vi "modbus Ref MCS .vi"() -> (4 "OffCoil":T3, 6 "On Coil":T2, 10 "Temp":T1)   [LabVIEW 2025]
uses:
  <vilib>/Modbus/master/Modbus Master.lvclass
  <vilib>/Analysis/NI_AALBase.lvlib
  <vilib>/Analysis/baseanly.llb/Mean (DBL).vi
  <vilib>/Modbus/master/Create Master Instance (TCP).vi
panel:
  in  "Boolean":bool
  out "TREES AVG array":dbl[](array[numeric])
  out "OD_Right side AVG distributed":dbl format="%0.2f"
  out "ON_Coil AVG distributed":dbl format="%0.2f"
  out "OFF_Coil AVG distributed":dbl format="%0.2f"
  out "AMB RIGHT":dbl[](array[numeric])
  out "ON-COIL 2":dbl[](array[numeric])
  out "OFF-COIL 2":dbl[](array[numeric])
  out "error out":errorcluster
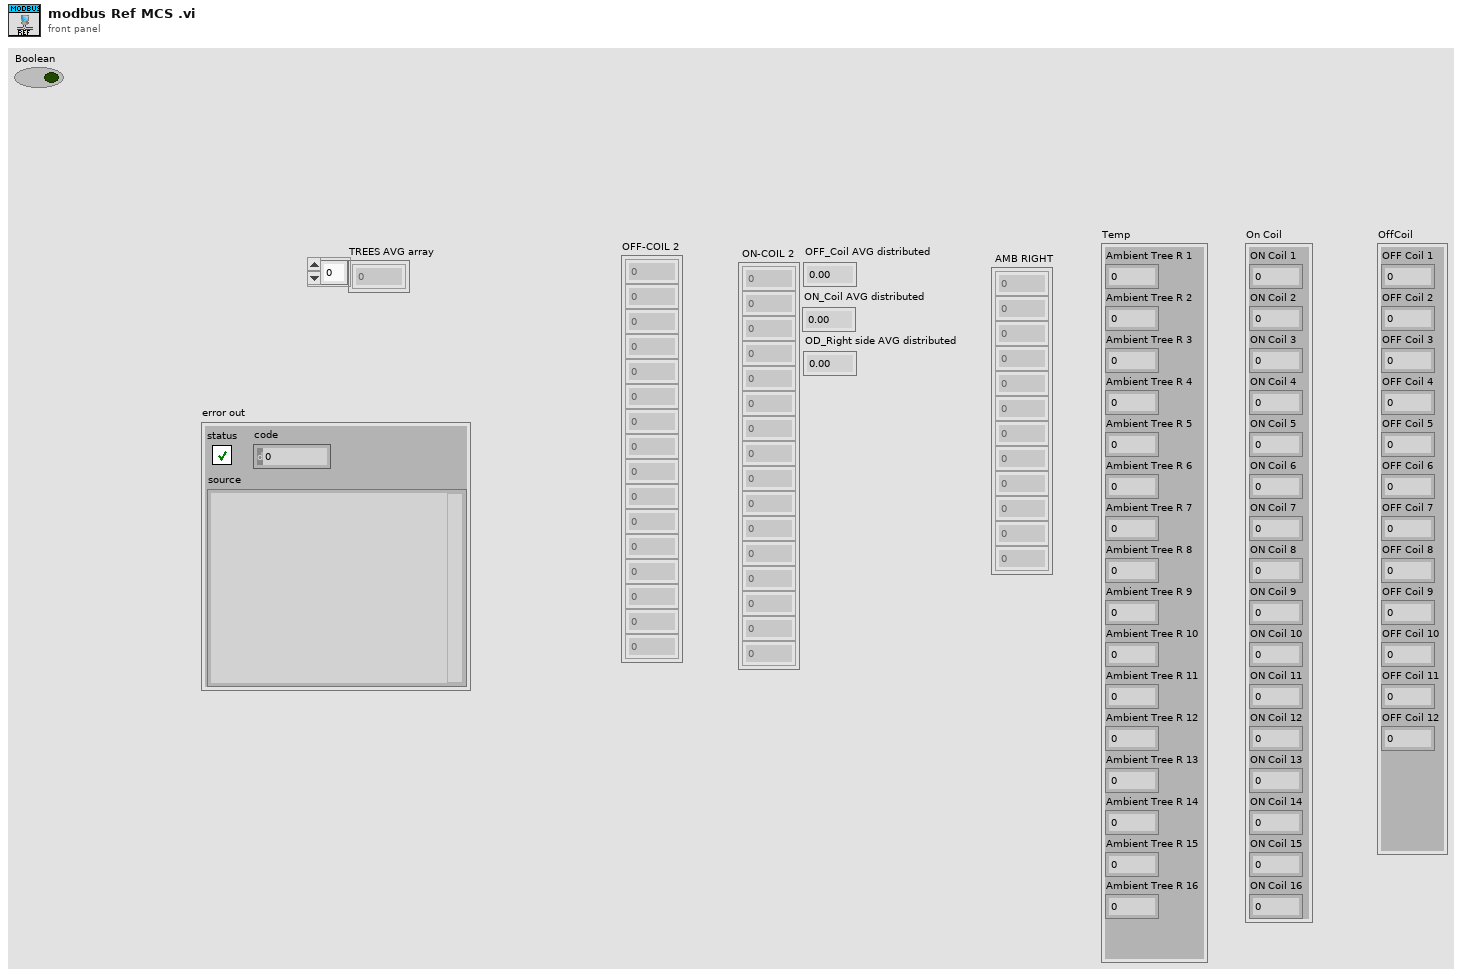
[diagram p1: front panel]
types:
  T1 = cluster{"Ambient Tree R 1":dbl, "Ambient Tree R 2":dbl, "Ambient Tree R 3":dbl, "Ambient Tree R 4":dbl, "Ambient Tree R 5":dbl, "Ambient Tree R 6":dbl, "Ambient Tree R 7":dbl, "Ambient Tree R 8":dbl, "Ambient Tree R 9":dbl, "Ambient Tree R 10":dbl, "Ambient Tree R 11":dbl, "Ambient Tree R 12":dbl, "Ambient Tree R 13":dbl, "Ambient Tree R 14":dbl, "Ambient Tree R 15":dbl, "Ambient Tree R 16":dbl}
  T2 = cluster{"ON Coil 1":dbl, "ON Coil 2":dbl, "ON Coil 3":dbl, "ON Coil 4":dbl, "ON Coil 5":dbl, "ON Coil 6":dbl, "ON Coil 7":dbl, "ON Coil 8":dbl, "ON Coil 9":dbl, "ON Coil 10":dbl, "ON Coil 11":dbl, "ON Coil 12":dbl, "ON Coil 13":dbl, "ON Coil 14":dbl, "ON Coil 15":dbl, "ON Coil 16":dbl}
  T3 = cluster{"OFF Coil 1":dbl, "OFF Coil 2":dbl, "OFF Coil 3":dbl, "OFF Coil 4":dbl, "OFF Coil 5":dbl, "OFF Coil 6":dbl, "OFF Coil 7":dbl, "OFF Coil 8":dbl, "OFF Coil 9":dbl, "OFF Coil 10":dbl, "OFF Coil 11":dbl, "OFF Coil 12":dbl}
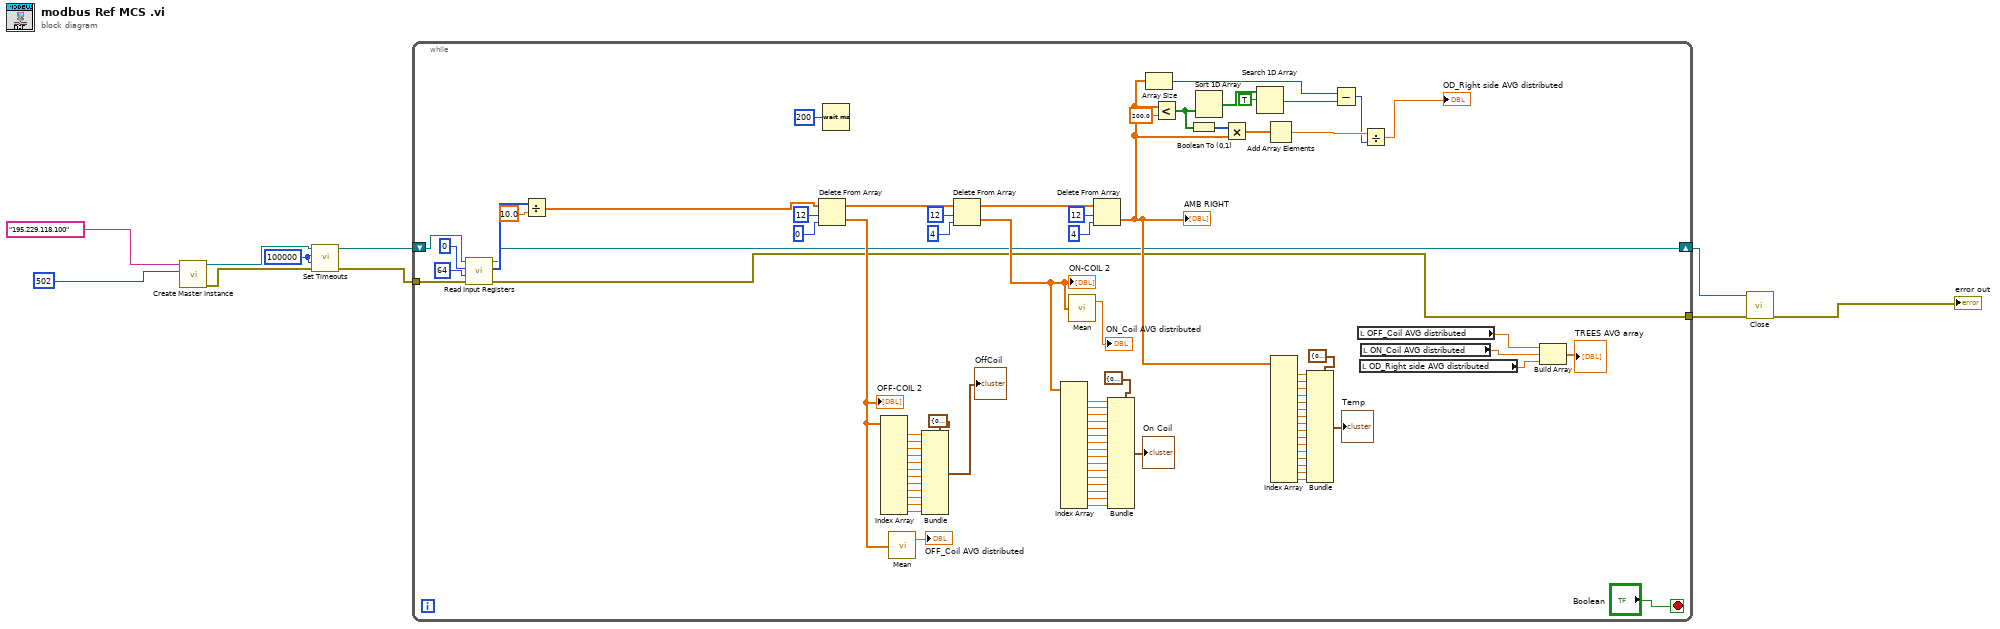
[diagram p0: block diagram]
diagram:
  w4 = 100000 ("read operation timeout (ms)")
  n1 = call-poly <vilib>:"Create Master Instance.vi"("port (502)"=u16 502, "address"="195.229.118.100") -> ("error out"=w5:errorcluster, "TCP master instance"=w6:refnum<class "Modbus Master.lvclass">)  [unwired: 8 in]
  n2 = call <vilib>:"Set Timeouts.vi"("error in (no error)"=w5, "write operation timeout (ms)"=w4, "read operation timeout (ms)"=w4, "Modbus master in"=w6) -> ("error out"=w10:errorcluster, "Modbus master out"=w9:refnum<class "Modbus Master.lvclass">)  [unwired: 6 in]
  n3 = while {
    tunnel: w10 -> [w20]
    tunnel: [w13] -> w2
    shift-right: [w12] -> w1
    shift-left: w9 -> [w19]
    stop <- "Boolean" stop-if-true
    n4 = call-dynamic "Read Input Registers.vi"("error in (no error)"=w20, "number of input registers"=u16 64, "starting address"=u16 0, "Modbus master in"=w19) -> ("error out"=w13:errorcluster, "register values"=w17:u16[], "Modbus master out"=w12:refnum<class "Modbus Master.lvclass">)  [unwired: 5 in]
    n5 = Divide(x=w17, y=10.0) -> (x/y=w21:dbl[])
    n6 = Delete From Array(array=w21, length=12, index=0) -> (deleted portion=w89:dbl[], array with subset deleted=w95:dbl[])
    "OFF-COIL 2" <- w89
    n7 = Wait (ms)(milliseconds to wait=u32 200) -> ()  [unwired: 1 out]
    n8 = Index Array(array=w89) -> (element #1=w87:dbl, element #2=w86:dbl, element #3=w85:dbl, element #4=w84:dbl, element #5=w83:dbl, element #6=w82:dbl, element #7=w81:dbl, element #8=w80:dbl, element #9=w79:dbl, element #10=w78:dbl, element #11=w77:dbl, element #12=w76:dbl)  [unwired: 12 in]
    n9 = call-poly <vilib>:"Mean.vi"("X"=w89) -> ("mean"=→"OFF_Coil AVG distributed":dbl)  [unwired: 1 out]
    n10 = Bundle(cluster=T3 {"OFF Coil 1"=0.0, "OFF Coil 2"=0.0, "OFF Coil 3"=0.0, "OFF Coil 4"=0.0, "OFF Coil 5"=0.0, "OFF Coil 6"=0.0, "OFF Coil 7"=0.0, "OFF Coil 8"=0.0, "OFF Coil 9"=0.0, "OFF Coil 10"=0.0, "OFF Coil 11"=0.0, "OFF Coil 12"=0.0}, "OFF Coil 1"=w87, "OFF Coil 2"=w86, "OFF Coil 3"=w85, "OFF Coil 4"=w84, "OFF Coil 5"=w83, "OFF Coil 6"=w82, "OFF Coil 7"=w81, "OFF Coil 8"=w80, "OFF Coil 9"=w79, "OFF Coil 10"=w78, "OFF Coil 11"=w77, "OFF Coil 12"=w76) -> (→"OffCoil":T3)
    n11 = Delete From Array(array=w95, length=12, index=4) -> (deleted portion=w74:dbl[], array with subset deleted=w92:dbl[])
    "ON-COIL 2" <- w74
    n12 = Index Array(array=w74) -> (element #1=w72:dbl, element #2=w71:dbl, element #3=w70:dbl, element #4=w69:dbl, element #5=w68:dbl, element #6=w67:dbl, element #7=w66:dbl, element #8=w65:dbl, element #9=w64:dbl, element #10=w63:dbl, element #11=w62:dbl, element #12=w61:dbl, element #13=w60:dbl, element #14=w59:dbl, element #15=w58:dbl, element #16=w57:dbl)  [unwired: 16 in]
    n13 = call-poly <vilib>:"Mean.vi"("X"=w74) -> ("mean"=→"ON_Coil AVG distributed":dbl)  [unwired: 1 out]
    n14 = Delete From Array(array=w92, length=12, index=4) -> (deleted portion=w28:dbl[])  [unwired: 1 out]
    "AMB RIGHT" <- w28
    n15 = Bundle(cluster=T2 {"ON Coil 1"=0.0, "ON Coil 2"=0.0, "ON Coil 3"=0.0, "ON Coil 4"=0.0, "ON Coil 5"=0.0, "ON Coil 6"=0.0, "ON Coil 7"=0.0, "ON Coil 8"=0.0, "ON Coil 9"=0.0, "ON Coil 10"=0.0, "ON Coil 11"=0.0, "ON Coil 12"=0.0, "ON Coil 13"=0.0, "ON Coil 14"=0.0, "ON Coil 15"=0.0, "ON Coil 16"=0.0}, "ON Coil 1"=w72, "ON Coil 2"=w71, "ON Coil 3"=w70, "ON Coil 4"=w69, "ON Coil 5"=w68, "ON Coil 6"=w67, "ON Coil 7"=w66, "ON Coil 8"=w65, "ON Coil 9"=w64, "ON Coil 10"=w63, "ON Coil 11"=w62, "ON Coil 12"=w61, "ON Coil 13"=w60, "ON Coil 14"=w59, "ON Coil 15"=w58, "ON Coil 16"=w57) -> (→"On Coil":T2)
    n16 = Array Size(array=w28) -> (size(s)=w30:i32)
    n17 = Less?(x=w28, y=200.0) -> (x < y?=w27:bool[])
    n18 = Boolean To (0,1)(Boolean=w27) -> (0, 1=w26:i16[])
    n19 = Sort 1D Array(array=w27) -> (sorted array=w32:bool[])
    n20 = Multiply(x=w26, y=w28) -> (x*y=w25:dbl[])
    n21 = Search 1D Array(1D array=w32, element=TRUE) -> (index of element=w29:i32)  [unwired: 1 in]
    n22 = Add Array Elements(numeric array=w25) -> (sum=w24:dbl)
    n23 = Index Array(array=w28) -> (element #1=w54:dbl, element #2=w53:dbl, element #3=w52:dbl, element #4=w51:dbl, element #5=w50:dbl, element #6=w49:dbl, element #7=w48:dbl, element #8=w47:dbl, element #9=w46:dbl, element #10=w45:dbl, element #11=w44:dbl, element #12=w43:dbl, element #13=w42:dbl, element #14=w41:dbl, element #15=w40:dbl, element #16=w39:dbl)  [unwired: 16 in]
    n24 = Bundle(cluster=T1 {"Ambient Tree R 1"=0.0, "Ambient Tree R 2"=0.0, "Ambient Tree R 3"=0.0, "Ambient Tree R 4"=0.0, "Ambient Tree R 5"=0.0, "Ambient Tree R 6"=0.0, "Ambient Tree R 7"=0.0, "Ambient Tree R 8"=0.0, "Ambient Tree R 9"=0.0, "Ambient Tree R 10"=0.0, "Ambient Tree R 11"=0.0, "Ambient Tree R 12"=0.0, "Ambient Tree R 13"=0.0, "Ambient Tree R 14"=0.0, "Ambient Tree R 15"=0.0, "Ambient Tree R 16"=0.0}, "Ambient Tree R 1"=w54, "Ambient Tree R 2"=w53, "Ambient Tree R 3"=w52, "Ambient Tree R 4"=w51, "Ambient Tree R 5"=w50, "Ambient Tree R 6"=w49, "Ambient Tree R 7"=w48, "Ambient Tree R 8"=w47, "Ambient Tree R 9"=w46, "Ambient Tree R 10"=w45, "Ambient Tree R 11"=w44, "Ambient Tree R 12"=w43, "Ambient Tree R 13"=w42, "Ambient Tree R 14"=w41, "Ambient Tree R 15"=w40, "Ambient Tree R 16"=w39) -> (→"Temp":T1)
    n25 = Subtract(x=w30, y=w29) -> (x-y=w23:i32)
    n26 = local read "OFF_Coil AVG distributed"() -> (w37:dbl)
    n27 = local read "OD_Right side AVG distributed"() -> (w35:dbl)
    n28 = local read "ON_Coil AVG distributed"() -> (w36:dbl)
    n29 = Divide(x=w24, y=w23) -> (x/y=→"OD_Right side AVG distributed":dbl)
    n30 = Build Array(w37, w36, w35) -> (→"TREES AVG array":dbl[])
  }
  n31 = call-dynamic "Close.vi"("error in (no error)"=w2, "Modbus master in"=w1) -> ("error out"=→"error out":errorcluster)  [unwired: 9 in]
